vi "VarexImager.vi"() -> ()   [LabVIEW 2025]
uses:
  typedef/fpscontrol.ctl
  <vilib>/vision/Image Controls.llb/IMAQ Image.ctl
  f14c558d-97a3-4ea9-8fc3-abe8e6238f6d.vi
  5a56aa01-388b-4886-999b-9eea1f9a46b5.vi
  VarexWrapper.lvlib
panel:
  out "Binning":i32
  out "displayTime (ms)":u32
  out "set fps status":i32
  out "integrationTimes":dbl[](array[numeric])
  out "gainCorr.Status":bool
  out "offsetCorr.Status":bool
  in  "Fps":T1 items=["25.0 fps (39.962 ms)", "20.0 fps (49.952 ms)", "10.0 fps (99.949 ms)", "5.0 fps (199.942 ms)", "3.0 fps (332.954 ms)", "2.0 fps (499.923 ms)", "1.0 fps (999.936 ms)", "0.7 fps (1399.955 ms)"]
  in  "Correction":bool
  in  "Load Correction":bool
  in  "Save Correction":bool
  out "acquisitionStatus":bool
  out "connStatus":bool
  out "Xlib Version":string
  out "Interface":string
  out "S. No":string
  in  "Ring Buffer Size":dbl
  in  "Frame Count":u32=100 caption="No of Frames for Calibration"
  out "Image":T2(plugin-control)
  out "Model":string
  out "Error out":errorcluster
  in  "Gain Correction":bool
  in  "Offset Correction":bool
  in  "Stop Acquisition":bool
  in  "Start Acquisition":bool
  in  "Disconnect":bool
  in  "Connect":bool
  # "Connection Control"
  # "Flat Field Correction"
  # "Acquisition Control"
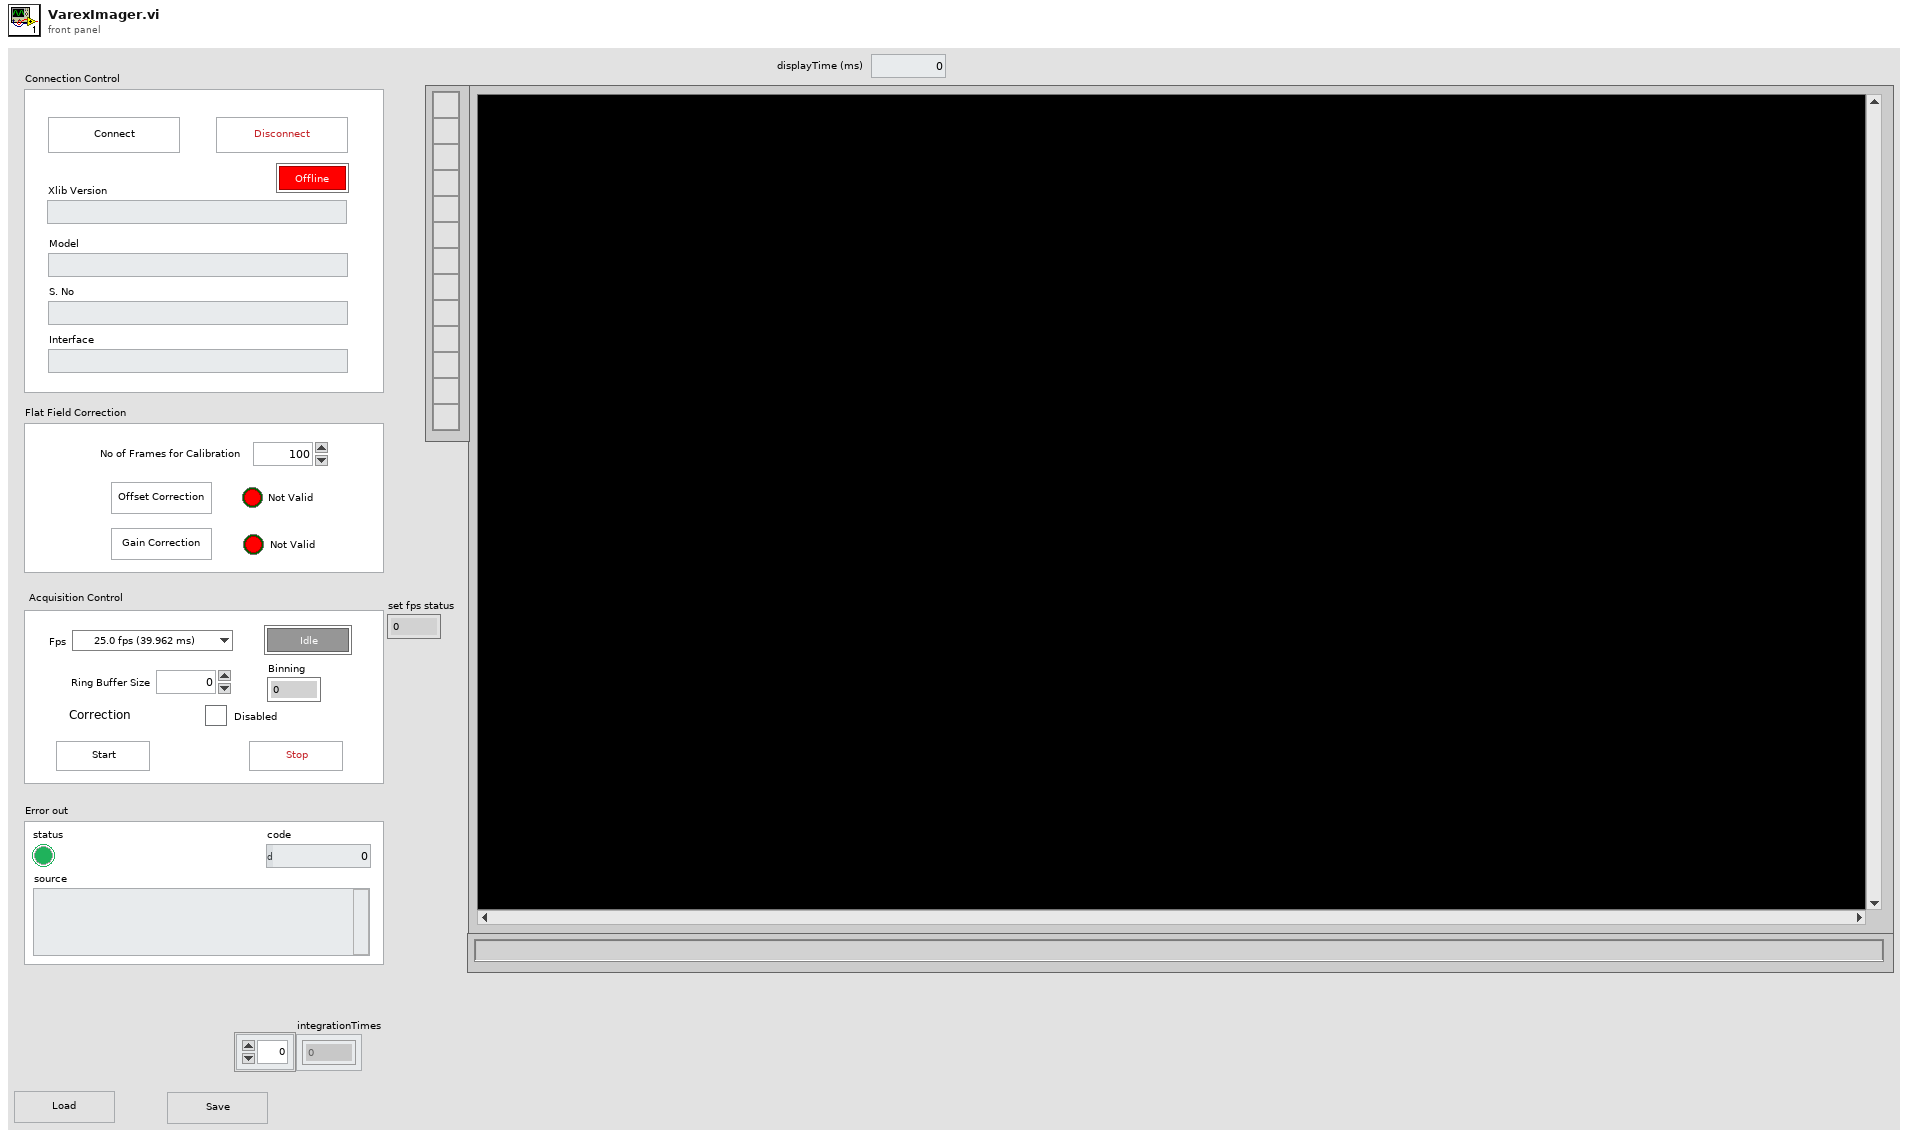
[diagram p1: front panel]
types:
  T1 = typedef "fpscontrol.ctl" = u16
  T2 = typedef "IMAQ Image.ctl" = refnum<image>
  T3 = cluster{"connStatus? (F)":bool, "acquire? (F)":bool, "img":T2, "gainMapPath":string, "offsetDataPath":string}
  T4 = typedef "Image Type" = u32
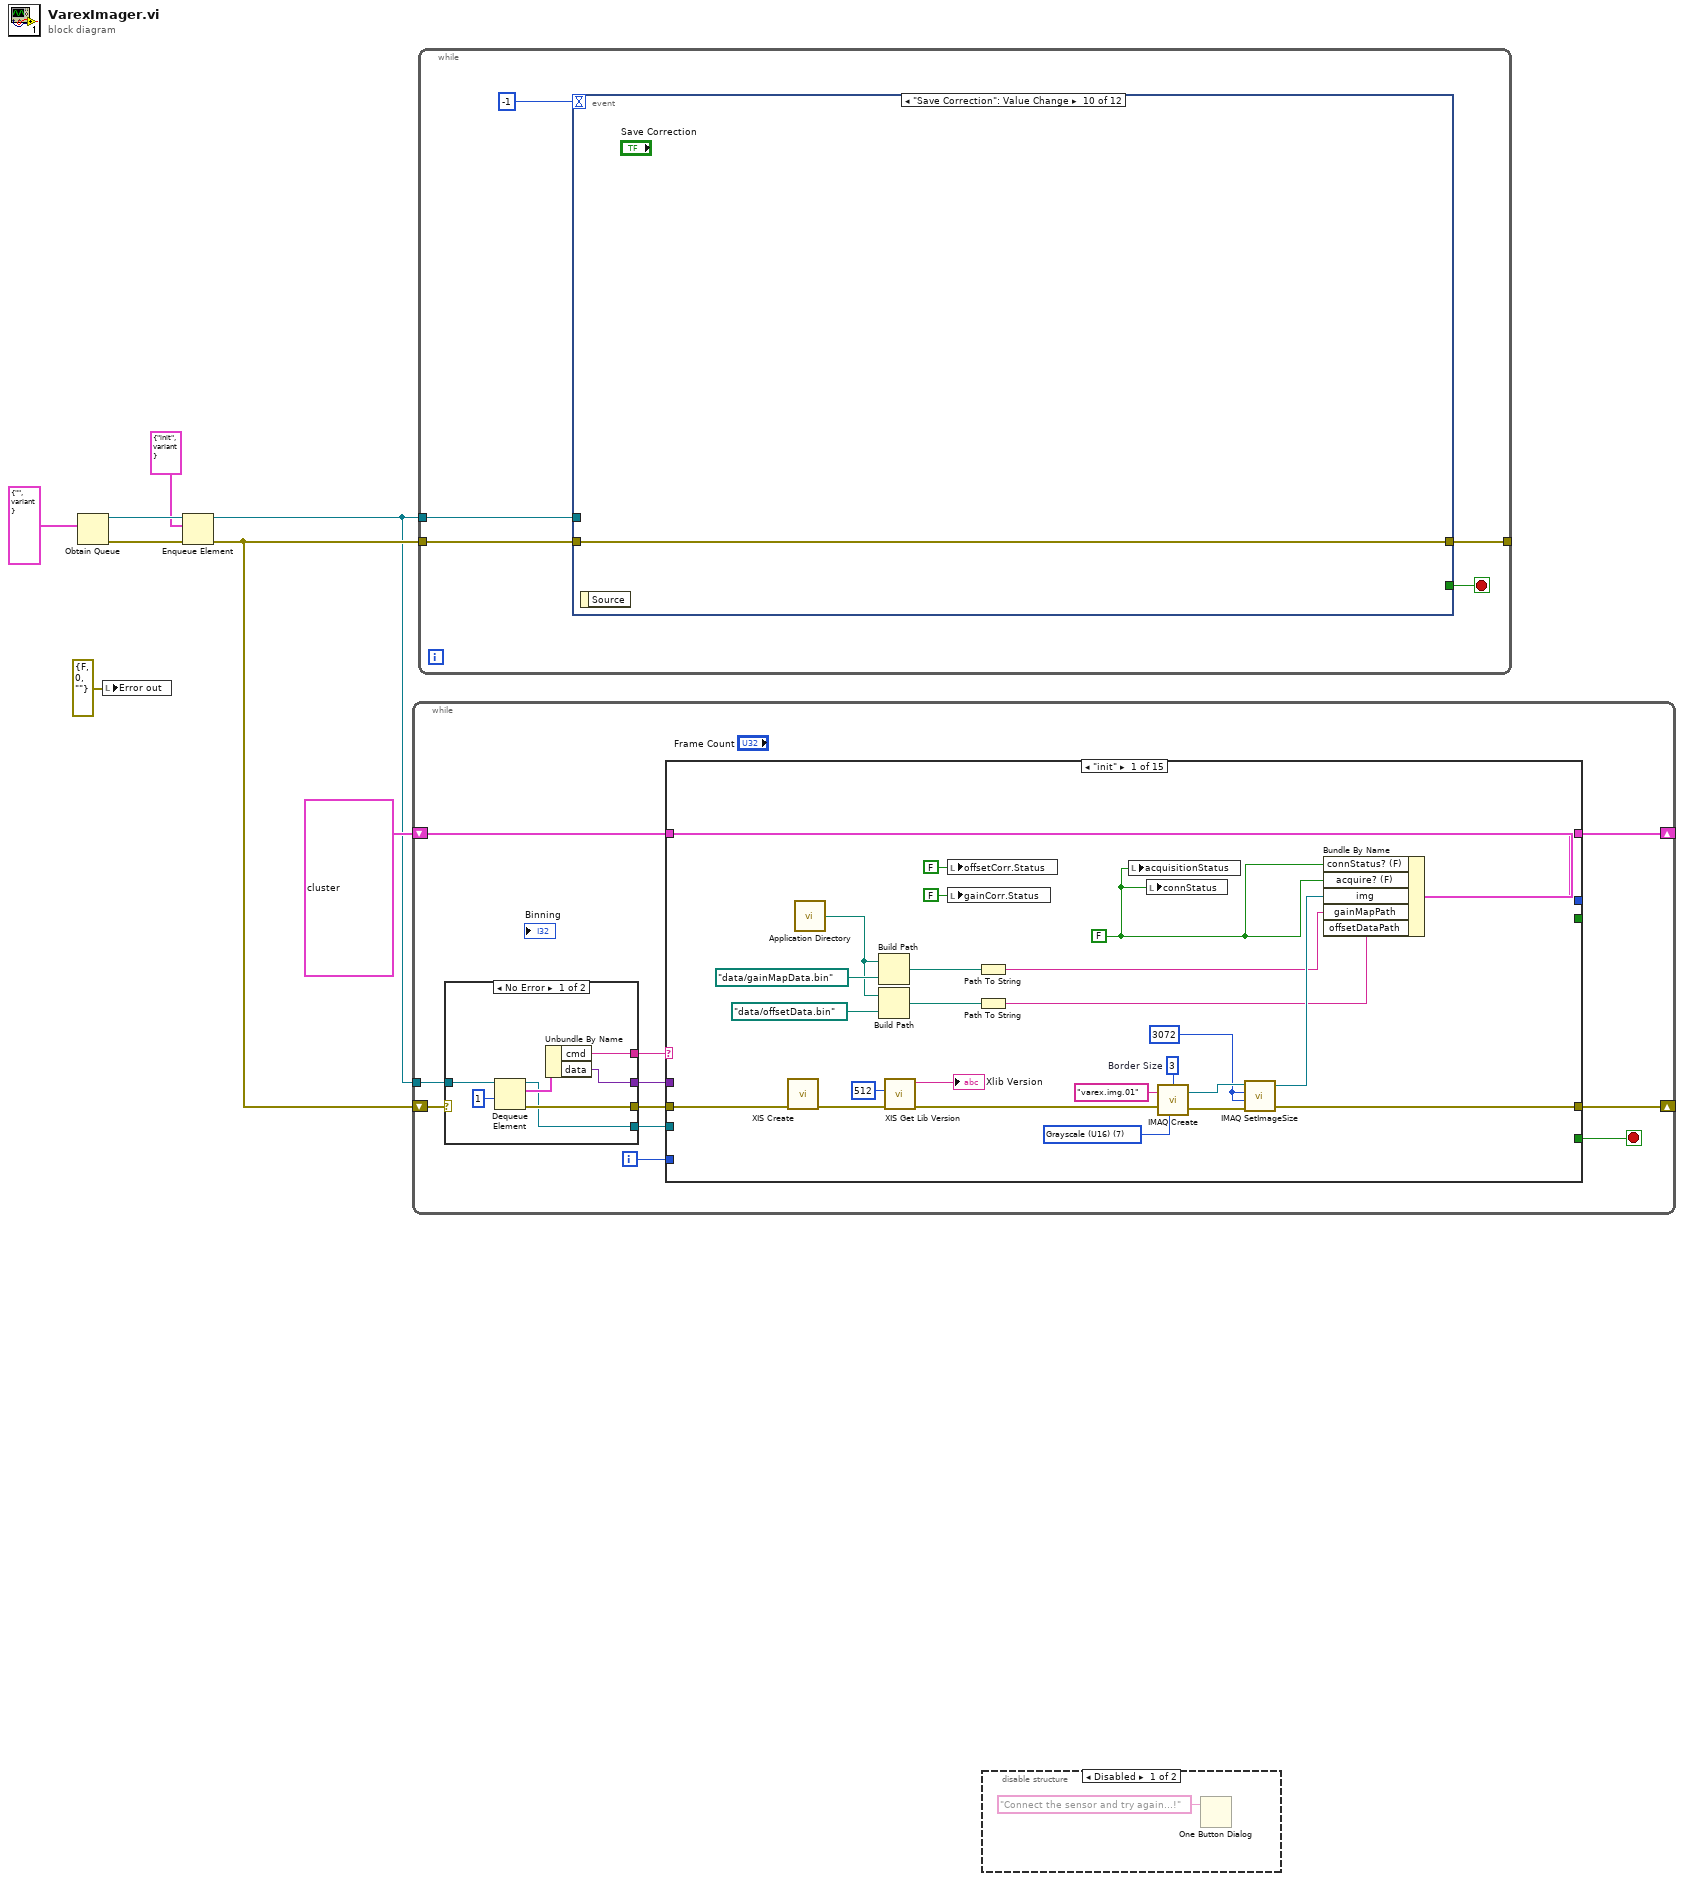
[diagram p0: block diagram]
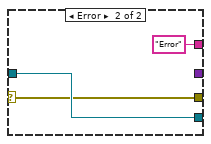
[diagram p3: hidden frame]
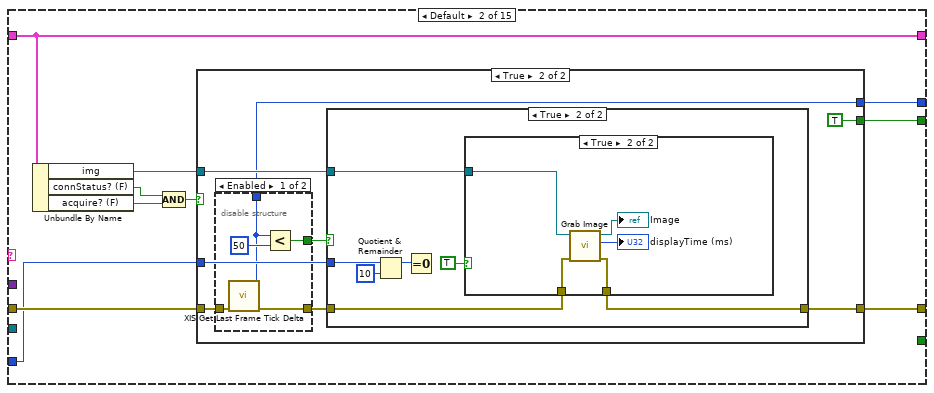
[diagram p4: hidden frame]
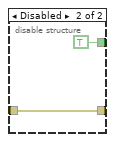
[diagram p6: hidden frame]
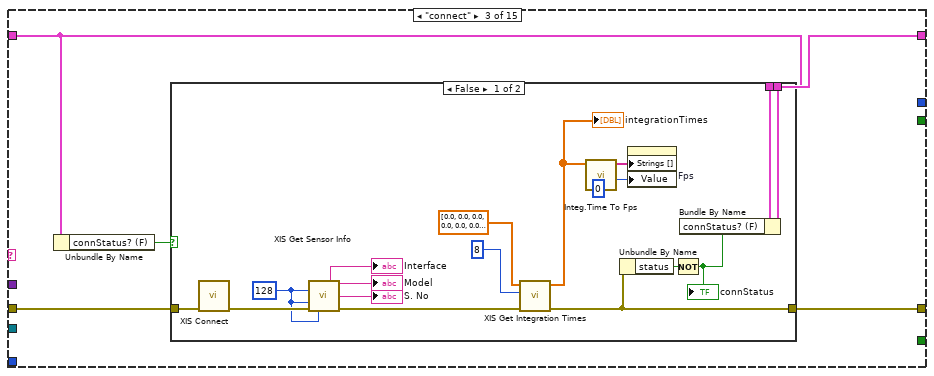
[diagram p9: hidden frame]
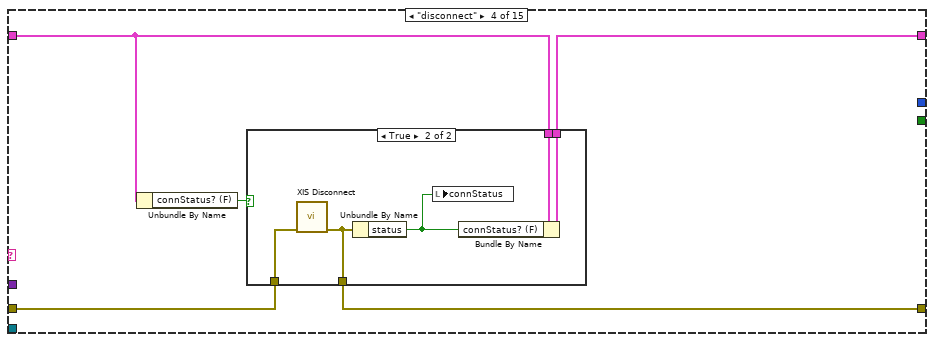
[diagram p11: hidden frame]
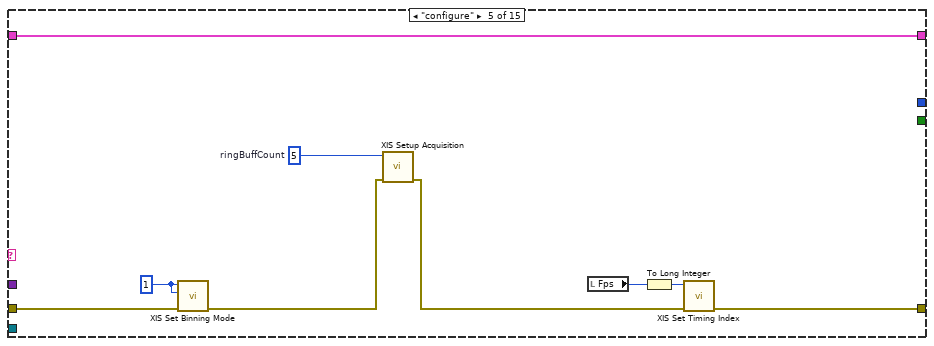
[diagram p13: hidden frame]
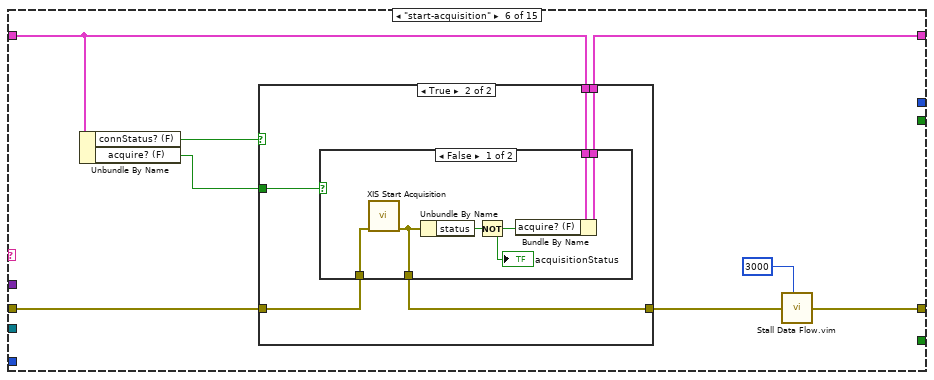
[diagram p14: hidden frame]
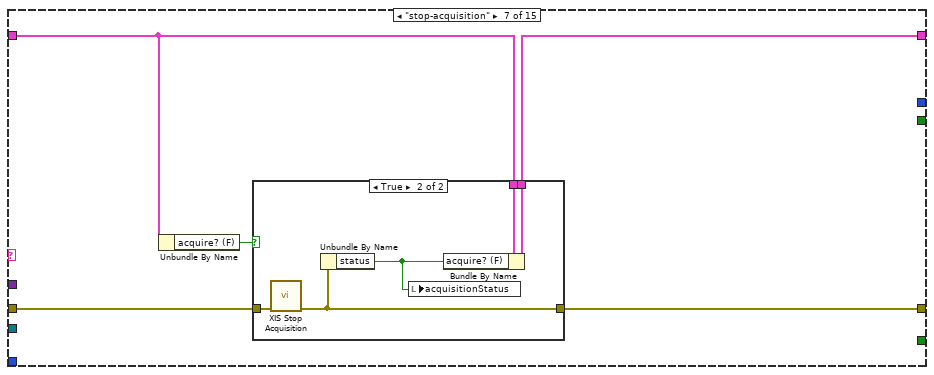
[diagram p17: hidden frame]
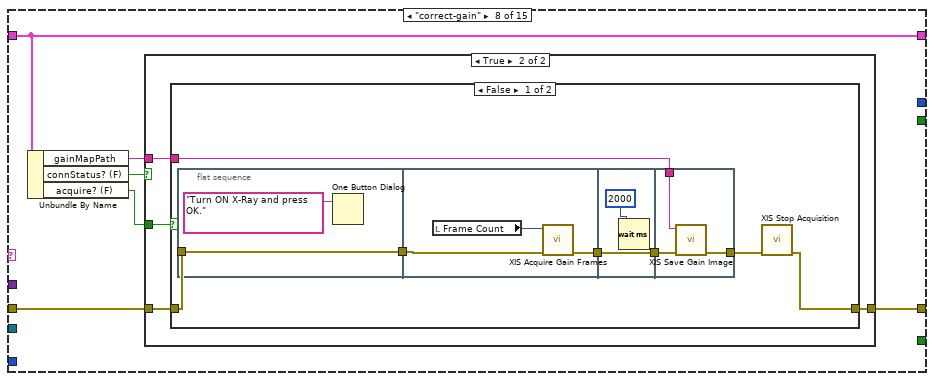
[diagram p19: hidden frame]
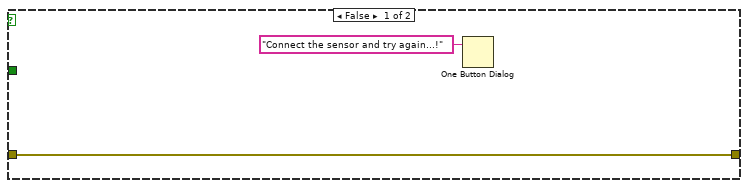
[diagram p20: hidden frame]
diagram:
  n1 = Obtain Queue(element data type=cluster{"cmd":string, "data":variant} {"cmd"="", "data"=variant}) -> (queue out=w4:refnum<queue>, error out=w7:errorcluster)  [unwired: 4 in, 1 out]
  n2 = local write "Error out"(errorcluster {"status"=FALSE, "code"=0, "source"=""} ("Error out")) -> ()
  n3 = Enqueue Element(queue=w4, element=cluster{"cmd":string, "data":variant} {"cmd"="init", "data"=variant}, error in (no error)=w7) -> (queue out=w3:refnum<queue>, error out=w5:errorcluster)  [unwired: 1 in, 1 out]
  n4 = while {
    tunnel: w3 -> [w19]
    shift-right: [w17] -> _
    shift-left: w5 -> [w16]
    shift-right: [w11] -> _
    shift-left: T3 {"connStatus? (F)"=FALSE, "acquire? (F)"=FALSE, "img"=refnum, "gainMapPath"="", "offsetDataPath"=""} -> [w12]
    i -> [w9]
    stop <- w10 stop-if-true
    n5 = case shown="No Error" w16 {
      selector: w16 -> [_ w28]
      tunnel: w19 -> [w26 w29]
      tunnel: [w25 w28] -> w18
      tunnel: [w23 w29] -> w15
      tunnel: [w22 "Error" ("cmd")] -> w14
      tunnel: [w21 _] -> w13
      frame No Error {
        n6 = Dequeue Element(queue=w26, timeout in ms (-1)=1) -> (queue out=w23:refnum<queue>, element=w24:cluster{"cmd":string, "data":variant}, error out=w25:errorcluster)  [unwired: 1 in, 1 out]
        n7 = Unbundle By Name(w24) -> ("cmd"=w22:string, "data"=w21:variant)
      }
      frame Error {
      }
    }
    n8 = case shown="\"init\"" w14 {
      tunnel: w18 -> [w52 w63 w99 w123 w138 w146 w167 w180 w211 w245 w254 w259 w265 w267 w275]
      tunnel: [w44 w62 w98 w122 w134 w141 w166 w179 w210 w243 w253 w257 w263 w266 w276] -> w17
      tunnel: w15 -> [_ _ _ _ _ _ _ _ _ _ _ _ _ _ _]
      tunnel: w13 -> [_ _ _ _ _ _ _ _ _ _ _ _ _ _ _]
      tunnel: w12 -> [w50 w64 w96 w120 w137 w143 w164 w178 w209 w244 w248 w258 w264 w268 w272]
      tunnel: [w41 w64 w97 w121 w137 w142 w163 w178 w209 w244 w248 w258 w264 w268 w272] -> w11
      tunnel: [_ _ _ _ _ _ _ _ _ _ _ _ _ _ TRUE] -> w10
      tunnel: w9 -> [_ w57 _ _ _ _ _ _ _ _ _ _ _ _ _]
      tunnel: [_ w56 _ _ _ _ _ _ _ _ _ _ _ _ _] -> _
      tunnel: [_ w55 _ _ _ _ _ _ _ _ _ _ _ _ _] -> _
      frame "init" {
        w39 = FALSE ("connStatus? (F)")
        w47 = 3  # Border Size
        w48 = 3072 ("X Resolution")
        w43 = T4 7 items=["Grayscale (U8)", "Grayscale (I16)", "Grayscale (SGL)", "Complex (CSG)", "RGB (U32)", "HSL (U32)", "RGB (U64)", "Grayscale (U16)"] ("Image Type")
        n9 = call "XIS Create.vi"("error in (no error)"=w52) -> ("error out"=w54:errorcluster)  [unwired: 9 in, 1 out]
        n10 = call <vilib>:"Application Directory.vi"() -> ("Application Directory"=w37:path)
        n11 = Build Path(base path=w37, name or relative path=path "data/gainMapData.bin") -> (appended path=w35:path)
        n12 = Build Path(base path=w37, name or relative path=path "data/offsetData.bin") -> (appended path=w34:path)
        n13 = call "XIS Get Lib Version.vi"("error in (no error)"=w54, "bufferSize"=512) -> ("error out"=w45:errorcluster, "buffer out"=→"Xlib Version":string)  [unwired: 7 in, 1 out]
        n14 = local write "offsetCorr.Status"(FALSE ("offsetCorr.Status")) -> ()
        n15 = local write "gainCorr.Status"(FALSE ("gainCorr.Status")) -> ()
        n16 = Path To String(path=w35) -> (string=w33:string)
        n17 = Path To String(path=w34) -> (string=w32:string)
        n18 = local write "acquisitionStatus"(w39) -> ()
        n19 = local write "connStatus"(w39) -> ()
        n20 = call "IMAQ Create"("Border Size"=w47, "Image Name"="varex.img.01", "Image Type"=w43, "error in (no error)"=w45) -> ("New Image"=w49:T2, "error out"=w46:errorcluster)  [unwired: 1 in]
        n21 = call "IMAQ SetImageSize"("error in (no error)"=w46, "Y Resolution"=w48, "X Resolution"=w48, "Image"=w49) -> ("error out"=w44:errorcluster, "Image Out"=w40:T2)  [unwired: 1 in]
        n22 = Bundle By Name(cluster=w50, "connStatus? (F)"=w39, "acquire? (F)"=w39, "img"=w40, "gainMapPath"=w33, "offsetDataPath"=w32) -> (w41:T3)
      }
      frame Default {
        n23 = Unbundle By Name(w64) -> ("img"=w58:T2, "connStatus? (F)"=w61:bool, "acquire? (F)"=w60:bool)
        n24 = Compound Arithmetic op=AND(w61, w60) -> (w59:bool)
        n25 = case shown="True" w59 {
          tunnel: w63 -> [w65 w71]
          tunnel: [w65 w73] -> w62
          tunnel: w58 -> [_ w72]
          tunnel: w57 -> [_ w69]
          tunnel: [_ w68] -> w56
          tunnel: [_ TRUE] -> w55
          frame False {
          }
          frame True {
            n26 = disable-structure shown="Enabled" {
              disable-tunnel: w71 -> [w78 w80]
              disable-tunnel: [w77 w80] -> w70
              disable-tunnel: [w75 TRUE] -> w66
              disable-tunnel: [w74 _] -> w68
              frame Enabled {
                n27 = call "XIS Get Last Frame Tick Delta.vi"("error in (no error)"=w78) -> ("error out"=w77:errorcluster, "function return"=w74:i32)  [unwired: 9 in]
                n28 = Less?(x=w74, y=50) -> (x < y?=w75:bool)
              }
              frame Disabled {
              }
            }
            n29 = case shown="True" w66 {
              tunnel: w70 -> [w81 w88]
              tunnel: [w81 w87] -> w73
              tunnel: w72 -> [_ w86]
              tunnel: w69 -> [_ w85]
              frame False {
                # "100 ms need to be changed based on the fps."
                # "Grabber is stabilizing..."
              }
              frame True {
                n30 = Quotient & Remainder(x=w85, y=10) -> (x-y*floor(x/y)=w84:i32)  [unwired: 1 out]
                n31 = Equal To 0?(x=w84) -> ()  [unwired: 1 out]
                n32 = case shown="True" TRUE {
                  tunnel: w88 -> [w89 w94]
                  tunnel: [w89 w92] -> w87
                  tunnel: w86 -> [_ w93]
                  frame False {
                  }
                  frame True {
                    n33 = call "Grab Image.vi"("error in (no error)"=w94, "Refnum in"=w93) -> ("error out"=w92:errorcluster, "displayTime"=→"displayTime (ms)":u32, "Refnum out"=→"Image":T2)  [unwired: 7 in]
                  }
                }
              }
            }
          }
        }
      }
      frame "connect" {
        n34 = Unbundle By Name(w96) -> ("connStatus? (F)"=w95:bool)
        n35 = case shown="False" w95 {
          tunnel: w99 -> [w114 w117]
          tunnel: [w105 w117] -> w98
          tunnel: w96 -> [w110 w118]
          tunnel: [w109 w118] -> w97
          frame False {
            w115 = 128 ("modelSize")
            n36 = call "XIS Connect.vi"("error in (no error)"=w114) -> ("error out"=w116:errorcluster)  [unwired: 9 in, 1 out]
            n37 = call "XIS Get Sensor Info.vi"("modelSize"=w115, "serialNumberSize"=w115, "error in (no error)"=w116, "channelTypeSize"=w115) -> ("channelType out"=→"Interface":string, "model out"=→"Model":string, "serialNumber out"=→"S. No":string, "error out"=w108:errorcluster)  [unwired: 7 in, 1 out]
            n38 = call "XIS Get Integration Times.vi"("error in (no error)"=w108, "count"=8, "timesArray"=dbl[] [0.0, 0.0, 0.0, 0.0, 0.0, 0.0, 0.0, 0.0]) -> ("error out"=w105:errorcluster, "timesArray out"=w102:dbl[])  [unwired: 5 in, 2 out]
            "integrationTimes" <- w102
            n39 = call "Integ.Time To Fps.vi"("integrationTimes (us)"=w102) -> ("fps string"=w101:string[])  [unwired: 10 in]
            n40 = Unbundle By Name(w105) -> ("status"=w107:bool)
            n41 = property on="Fps" class="Ring (strict)"("Strings []"=w101, "Value"=u16 0) -> ()  [unwired: 2 in, 2 out]
            n42 = Not(x=w107) -> (.not. x?=w106:bool)
            "connStatus" <- w106
            n43 = Bundle By Name(cluster=w110, "connStatus? (F)"=w106) -> (w109:T3)
          }
          frame True {
          }
        }
      }
      frame "disconnect" {
        n44 = Unbundle By Name(w120) -> ("connStatus? (F)"=w119:bool)
        n45 = case shown="True" w119 {
          tunnel: w123 -> [w124 w130]
          tunnel: [w124 w127] -> w122
          tunnel: w120 -> [w125 w129]
          tunnel: [w125 w128] -> w121
          frame False {
          }
          frame True {
            n46 = call "XIS Disconnect.vi"("error in (no error)"=w130) -> ("error out"=w127:errorcluster)  [unwired: 9 in, 1 out]
            n47 = Unbundle By Name(w127) -> ("status"=w126:bool)
            n48 = local write "connStatus"(w126) -> ()
            n49 = Bundle By Name(cluster=w129, "connStatus? (F)"=w126) -> (w128:T3)
          }
        }
      }
      frame "configure" {
        w131 = 1 ("binningMode")
        w139 = 5  # ringBuffCount
        n50 = call "XIS Set Binning Mode.vi"("error in (no error)"=w138, "accumulated"=w131, "binningMode"=w131) -> ("error out"=w132:errorcluster)  [unwired: 7 in, 1 out]
        n51 = call "XIS Setup Acquisition.vi"("error in (no error)"=w132, "ringBuffCount"=w139) -> ("error out"=w135:errorcluster)  [unwired: 8 in, 1 out]
        n52 = local read "Fps"() -> (w133:T1)
        n53 = To Long Integer(number=w133) -> (32bit integer=w136:i32)
        n54 = call "XIS Set Timing Index.vi"("error in (no error)"=w135, "timingIndex"=w136) -> ("error out"=w134:errorcluster)  [unwired: 8 in, 1 out]
      }
      frame "start-acquisition" {
        n55 = Unbundle By Name(w143) -> ("connStatus? (F)"=w145:bool, "acquire? (F)"=w144:bool)
        n56 = case shown="True" w145 {
          tunnel: [w149 w154] -> w147
          tunnel: w146 -> [w149 w153]
          tunnel: w144 -> [_ w152]
          tunnel: w143 -> [w148 w151]
          tunnel: [w148 w150] -> w142
          frame False {
          }
          frame True {
            n57 = case shown="False" w152 {
              tunnel: [w157 w161] -> w154
              tunnel: w153 -> [w160 w161]
              tunnel: w151 -> [w159 w162]
              tunnel: [w158 w162] -> w150
              frame False {
                n58 = call "XIS Start Acquisition.vi"("error in (no error)"=w160) -> ("error out"=w157:errorcluster)  [unwired: 9 in, 1 out]
                n59 = Unbundle By Name(w157) -> ("status"=w156:bool)
                n60 = Not(x=w156) -> (.not. x?=w155:bool)
                "acquisitionStatus" <- w155
                n61 = Bundle By Name(cluster=w159, "acquire? (F)"=w155) -> (w158:T3)
              }
              frame True {
              }
            }
          }
        }
        n62 = call "Stall Data Flow.vim"("value in"=w147, "milliseconds to wait"=u32 3000) -> ("value out"=w141:errorcluster)  [unwired: 1 out]
      }
      frame "stop-acquisition" {
        n63 = Unbundle By Name(w164) -> ("acquire? (F)"=w165:bool)
        n64 = case shown="True" w165 {
          tunnel: w167 -> [w169 w174]
          tunnel: [w169 w171] -> w166
          tunnel: w164 -> [w168 w173]
          tunnel: [w168 w172] -> w163
          frame False {
          }
          frame True {
            n65 = call "XIS Stop Acquisition.vi"("error in (no error)"=w174) -> ("error out"=w171:errorcluster)  [unwired: 9 in, 1 out]
            n66 = Unbundle By Name(w171) -> ("status"=w170:bool)
            n67 = local write "acquisitionStatus"(w170) -> ()
            n68 = Bundle By Name(cluster=w173, "acquire? (F)"=w170) -> (w172:T3)
          }
        }
      }
      frame "correct-gain" {
        n69 = Unbundle By Name(w178) -> ("gainMapPath"=w175:string, "connStatus? (F)"=w177:bool, "acquire? (F)"=w176:bool)
        n70 = case shown="True" w177 {
          tunnel: w180 -> [w182 w186]
          tunnel: [w182 w185] -> w179
          tunnel: w176 -> [_ w184]
          tunnel: w175 -> [_ w183]
          frame False {
            n71 = One Button Dialog(message="Connect the sensor and try again...!") -> ()  [unwired: 1 in, 1 out]
          }
          frame True {
            n72 = case shown="False" w184 {
              tunnel: w186 -> [w192 w205]
              tunnel: [w187 w205] -> w185
              tunnel: w183 -> [w189 _]
              frame False {
                n73 = flat-sequence {
                  tunnel: w192 -> [w195]
                  tunnel: [w195] -> w193
                  tunnel: w193 -> [w198]
                  tunnel: [w196] -> w190
                  tunnel: [w200] -> w191
                  tunnel: w190 -> [w200]
                  tunnel: [w202] -> w188
                  tunnel: w191 -> [w203]
                  tunnel: w189 -> [w201]
                  frame #0 {
                    n74 = One Button Dialog(message="Turn ON X-Ray and press OK.") -> ()  [unwired: 1 in, 1 out]
                  }
                  frame #1 {
                    n75 = local read "Frame Count"() -> (w197:u32)
                    n76 = call "XIS Acquire Gain Frames.vi"("error in (no error)"=w198, "numFrames"=w197) -> ("error out"=w196:errorcluster)  [unwired: 8 in, 1 out]
                  }
                  frame #2 {
                    n77 = Wait (ms)(milliseconds to wait=u32 2000) -> ()  [unwired: 1 out]
                  }
                  frame #3 {
                    n78 = call "XIS Save Gain Image.vi"("error in (no error)"=w203, "filePath"=w201) -> ("error out"=w202:errorcluster)  [unwired: 8 in, 1 out]
                  }
                }
                n79 = call "XIS Stop Acquisition.vi"("error in (no error)"=w188) -> ("error out"=w187:errorcluster)  [unwired: 9 in, 1 out]
              }
              frame True {
                n80 = One Button Dialog(message="Turn OFF Acquisition and try again...!") -> ()  [unwired: 1 in, 1 out]
              }
            }
          }
        }
      }
      frame "correct-offset" {
        n81 = Unbundle By Name(w209) -> ("offsetDataPath"=w206:string, "connStatus? (F)"=w208:bool, "acquire? (F)"=w207:bool)
        n82 = case shown="True" w208 {
          tunnel: w211 -> [w213 w217]
          tunnel: [w213 w216] -> w210
          tunnel: w207 -> [_ w215]
          tunnel: w206 -> [_ w214]
          frame False {
            n83 = One Button Dialog(message="Connect the sensor and try again...!") -> ()  [unwired: 1 in, 1 out]
          }
          frame True {
            n84 = case shown="False" w215 {
              tunnel: w217 -> [w223 w236]
              tunnel: [w218 w236] -> w216
              tunnel: w214 -> [w219 _]
              frame False {
                n85 = flat-sequence {
                  tunnel: w223 -> [w226]
                  tunnel: [w226] -> w224
                  tunnel: w224 -> [w229]
                  tunnel: [w227] -> w220
                  tunnel: [w231] -> w221
                  tunnel: w220 -> [w231]
                  tunnel: [w232] -> w222
                  tunnel: w221 -> [w234]
                  tunnel: w219 -> [w233]
                  frame #0 {
                    n86 = One Button Dialog(message="Turn OFF X-Ray and press OK.") -> ()  [unwired: 1 in, 1 out]
                  }
                  frame #1 {
                    n87 = local read "Frame Count"() -> (w228:u32)
                    n88 = call "XIS Acquire Offset Frames.vi"("error in (no error)"=w229, "numFrames"=w228) -> ("error out"=w227:errorcluster)  [unwired: 8 in, 1 out]
                  }
                  frame #2 {
                    n89 = Wait (ms)(milliseconds to wait=u32 2000) -> ()  [unwired: 1 out]
                  }
                  frame #3 {
                    n90 = call "XIS Save Offset Image.vi"("error in (no error)"=w234, "filePath"=w233) -> ("error out"=w232:errorcluster)  [unwired: 8 in, 1 out]
                  }
                }
                n91 = call "XIS Stop Acquisition.vi"("error in (no error)"=w222) -> ("error out"=w218:errorcluster)  [unwired: 9 in, 1 out]
              }
              frame True {
                n92 = One Button Dialog(message="Turn OFF Acquisition and try again...!") -> ()  [unwired: 1 in, 1 out]
              }
            }
          }
        }
      }
      frame "check-correction-status" {
        n93 = call "XIS Is Correction Ready.vi"("error in (no error)"=w245) -> ("error out"=w243:errorcluster, "gainReady out"=w241:i32, "offsetReady out"=w242:i32)  [unwired: 7 in, 1 out]
        n94 = Equal To 0?(x=w242) -> (x = 0?=w240:bool)
        n95 = Equal To 0?(x=w241) -> (x = 0?=w239:bool)
        n96 = Not(x=w240) -> (.not. x?=→"offsetCorr.Status":bool)
        n97 = Not(x=w239) -> (.not. x?=→"gainCorr.Status":bool)
      }
      frame "enable-correction" {
        n98 = Unbundle By Name(w248) -> ("offsetDataPath"=w247:string, "gainMapPath"=w246:string)
        n99 = call "XIS Load Gain Image.vi"("error in (no error)"=w254, "filePath"=w246) -> ("error out"=w250:errorcluster)  [unwired: 8 in, 1 out]
        n100 = call "XIS Load Offset Image.vi"("error in (no error)"=w250, "filePath"=w247) -> ("error out"=w249:errorcluster)  [unwired: 8 in, 1 out]
        n101 = call "XIS Set Correction Enabled.vi"("error in (no error)"=w249, "enableGain"=1, "enableOffset"=1) -> ("error out"=w253:errorcluster)  [unwired: 7 in, 1 out]
      }
      frame "disable-correction" {
        n102 = call "XIS Set Correction Enabled.vi"("error in (no error)"=w259, "enableGain"=0, "enableOffset"=0) -> ("error out"=w257:errorcluster)  [unwired: 7 in, 1 out]
      }
      frame "set-integration-time" {
        n103 = local read "Fps"() -> (w262:T1)
        n104 = To Long Integer(number=w262) -> (32bit integer=w261:i32)
        n105 = call "XIS Set Timing Index.vi"("error in (no error)"=w265, "timingIndex"=w261) -> ("error out"=w263:errorcluster, "function return"=→"set fps status":i32)  [unwired: 8 in]
      }
      frame "error" {
        n106 = call <vilib>:"Clear Errors.vi"("error in (no error)"=w267) -> ("error out"=w266:errorcluster)  [unwired: 5 in, 1 out]
        "Error out" <- w267
      }
      frame "exit" {
        n107 = Unbundle By Name(w272) -> ("connStatus? (F)"=w270:bool, "acquire? (F)"=w271:bool)
        n108 = case shown="True" w271 {
          tunnel: w275 -> [w277 w279]
          tunnel: [w277 w278] -> w274
          frame False {
          }
          frame True {
            n109 = call "XIS Stop Acquisition.vi"("error in (no error)"=w279) -> ("error out"=w278:errorcluster)  [unwired: 9 in, 1 out]
          }
        }
        n110 = case shown="True" w270 {
          tunnel: w274 -> [w280 w282]
          tunnel: [w280 w281] -> w273
          frame False {
          }
          frame True {
            n111 = call "XIS Disconnect.vi"("error in (no error)"=w282) -> ("error out"=w281:errorcluster)  [unwired: 9 in, 1 out]
          }
        }
        n112 = call "XIS Destroy.vi"("error in (no error)"=w273) -> ("error out"=w276:errorcluster)  [unwired: 9 in, 1 out]
      }
    }
  }
  n113 = while {
    tunnel: w3 -> [w285]
    tunnel: w5 -> [w287]
    tunnel: [w286] -> _
    stop <- w283 stop-if-true
    n114 = event shown="[9] \"Save Correction\": Value Change" {
      selector: _ -> [_ _ _ _ _ _ _ _ _ _ _ _]
      dyn-events: _ -> [_ _ _ _ _ _ _ _ _ _ _ _]
      timeout: -1 -> [_ _ _ _ _ _ _ _ _ _ _ _]
      tunnel: w287 -> [w288 w295 w299 w303 w310 w321 w328 w334 w335 w336 w340 w349]
      tunnel: [w288 w291 w298 w302 w309 w324 w327 w331 w335 w336 w339 w348] -> w286
      tunnel: w285 -> [_ w294 w297 w301 w308 w319 w326 w330 _ _ w338 w347]
      tunnel: [_ _ _ _ _ _ _ TRUE _ _ _ _] -> w283
      event Timeout {
        n115 = event-data() -> ()  [unwired: 1 in, 3 out]
      }
      event "Connect": Value Change {
        n116 = event-data() -> ()  [unwired: 1 in, 1 out]
        n117 = Enqueue Element(queue=w294, element=cluster{"cmd":string, "data":variant} {"cmd"="connect", "data"=variant}, error in (no error)=w295) -> (queue out=w290:refnum<queue>, error out=w292:errorcluster)  [unwired: 1 in, 1 out]
        n118 = Enqueue Element(queue=w290, element=cluster{"cmd":string, "data":variant} {"cmd"="configure", "data"=variant}, error in (no error)=w292) -> (error out=w291:errorcluster)  [unwired: 1 in, 2 out]
      }
      event "Disconnect": Value Change {
        n119 = event-data() -> ()  [unwired: 1 in, 1 out]
        n120 = Enqueue Element(queue=w297, element=cluster{"cmd":string, "data":variant} {"cmd"="disconnect", "data"=variant}, error in (no error)=w299) -> (error out=w298:errorcluster)  [unwired: 1 in, 2 out]
      }
      event "Offset Correction": Value Change {
        # "correct-offset"
        n121 = event-data() -> ()  [unwired: 1 in, 1 out]
        n122 = for {
          tunnel: w301 -> [w305]
          tunnel: cluster{"cmd":string, "data":variant}[] [{"cmd"="correct-offset", "data"=variant}, {"cmd"="check-correction-status", "data"=variant}] ("element") -> [w304] mode=indexing
          shift-right: [w306] -> w302
          shift-left: w303 -> [w307]
          n123 = Enqueue Element(queue=w305, element=w304, error in (no error)=w307) -> (error out=w306:errorcluster)  [unwired: 1 in, 2 out]
        }
      }
      event "Gain Correction": Value Change {
        n124 = event-data() -> ()  [unwired: 1 in, 1 out]
        n125 = for {
          tunnel: w308 -> [w313]
          tunnel: cluster{"cmd":string, "data":variant}[] [{"cmd"="correct-gain", "data"=variant}, {"cmd"="check-correction-status", "data"=variant}] ("element") -> [w312] mode=indexing
          shift-right: [w314] -> w309
          shift-left: w310 -> [w315]
          n126 = Enqueue Element(queue=w313, element=w312, error in (no error)=w315) -> (error out=w314:errorcluster)  [unwired: 1 in, 2 out]
        }
      }
      event "Start Acquisition": Value Change {
        n127 = event-data() -> ()  [unwired: 1 in, 1 out]
        n128 = Enqueue Element(queue=w319, element=cluster{"cmd":string, "data":variant} {"cmd"="configure", "data"=variant}, error in (no error)=w321) -> (queue out=w316:refnum<queue>, error out=w320:errorcluster)  [unwired: 1 in, 1 out]
        n129 = call "Stall Data Flow.vim"("value in"=w320, "milliseconds to wait"=u32 1000) -> ("value out"=w318:errorcluster)  [unwired: 1 out]
        n130 = Enqueue Element(queue=w316, element=cluster{"cmd":string, "data":variant} {"cmd"="start-acquisition", "data"=variant}, error in (no error)=w318) -> (error out=w324:errorcluster)  [unwired: 1 in, 2 out]
      }
      event "Stop Acquisition": Value Change {
        n131 = event-data() -> ()  [unwired: 1 in, 1 out]
        n132 = Enqueue Element(queue=w326, element=cluster{"cmd":string, "data":variant} {"cmd"="stop-acquisition", "data"=variant}, error in (no error)=w328) -> (error out=w327:errorcluster)  [unwired: 1 in, 2 out]
      }
      event Panel Close? {
        n133 = event-data() -> ()  [unwired: 1 in, 1 out]
        n134 = Enqueue Element(queue=w330, element=cluster{"cmd":string, "data":variant} {"cmd"="exit", "data"=variant}, error in (no error)=w334) -> (error out=w331:errorcluster)  [unwired: 1 in, 2 out]
        n135 = event-data("Discard?"=TRUE) -> ()  [unwired: 1 in, 1 out]
      }
      event "Load Correction": Value Change {
        n136 = event-data() -> ()  [unwired: 1 in, 1 out]
      }
      event "Save Correction": Value Change {
        n137 = event-data() -> ()  [unwired: 1 in, 1 out]
      }
      event Value Change {
        n138 = event-data() -> ()  [unwired: 1 in, 1 out]
        n139 = Enqueue Element(queue=w338, element=cluster{"cmd":string, "data":variant} {"cmd"="set-integration-time", "data"=variant}, error in (no error)=w340) -> (error out=w339:errorcluster)  [unwired: 1 in, 2 out]
      }
      event "Correction": Value Change {
        n140 = event-data() -> ("NewVal"=w344:bool)  [unwired: 1 in]
        n141 = Select(t="enable-correction" ("cmd"), s=w344, f="disable-correction" ("cmd")) -> (s? t:f=w343:string)
        n142 = Bundle By Name(cluster=cluster{"cmd":string, "data":variant} {"cmd"="", "data"=variant} ("element"), "cmd"=w343) -> (w345:cluster{"cmd":string, "data":variant})
        n143 = Enqueue Element(queue=w347, element=w345, error in (no error)=w349) -> (error out=w348:errorcluster)  [unwired: 1 in, 2 out]
      }
    }
  }
  n144 = disable-structure shown="Disabled" {
    frame Disabled {
      n145 = One Button Dialog(message="Connect the sensor and try again...!") -> ()  [unwired: 1 in, 1 out]
    }
    frame Enabled {
    }
  }
